vi "nominal_data_source.create.vi"(8 "error in":errorcluster, 9 "Description":string, 10 "Name":string, 11 "Nominal Client in":refnum<class "Nominal Client.lvclass">) -> (0 "error out":errorcluster, 1 "Created Data Source":T1, 2 "rid":string, 3 "Nominal Client out":refnum<class "Nominal Client.lvclass">)   [LabVIEW 2020, in "Nominal Client.lvclass"]
doc: "Creates a data source.\n\nid -> Required\nA human readable identifier. Must be unique within an organization. If the ID is not unique, a timestamp will be added to the ID.\n\ndescription -> Optional"
uses:
  Nominal Client.lvclass
  609118db-7d9c-428b-a577-7bf67d0e67c4.vi
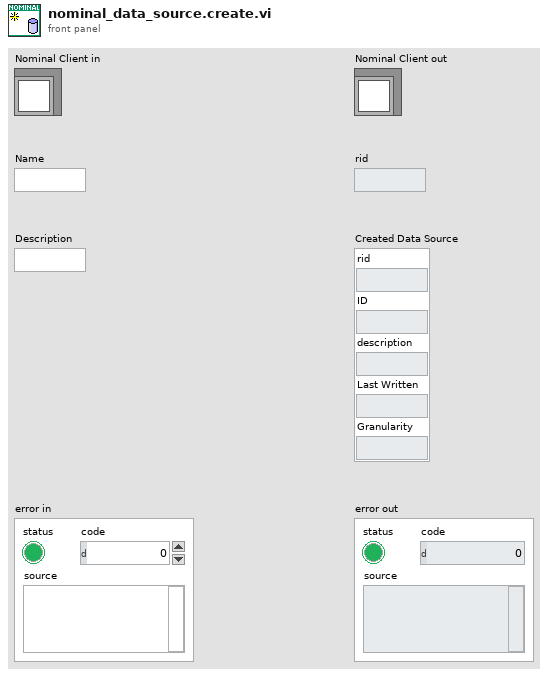
[diagram p1: front panel]
types:
  T1 = cluster{"rid":string, "ID":string, "description":string, "Last Written":string, "Granularity":string}
  T2 = cluster{"rid":string, "id":string, "description":string, "dataLastWrittenAt":string, "granularity":string}
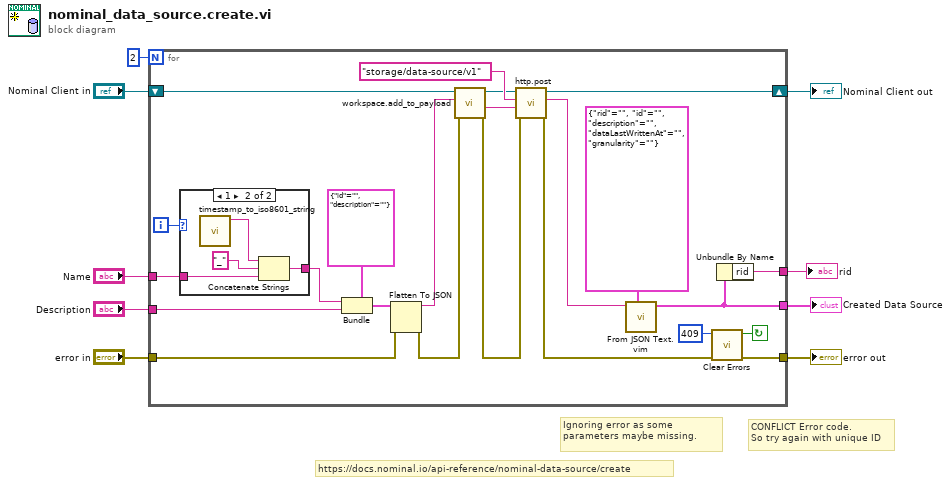
[diagram p0: block diagram]
diagram:
  # "CONFLICT Error code.\nSo try again with unique ID"
  # "Ignoring error as some parameters maybe missing."
  # "https://docs.nominal.io/api-reference/nominal-data-source/create"
  n1 = for {
    N: 2 -> [_]
    tunnel: "Name" -> [w21]
    tunnel: "Description" -> [w28]
    tunnel: [w24] -> w3
    tunnel: [w23] -> w2
    shift-right: [w32] -> w8
    shift-left: "Nominal Client in" -> [w15]
    tunnel: "error in" -> [w29]
    tunnel: [w17] -> w4
    i -> [w22]
    stop <- w16 continue-if-true
    n2 = case shown="1" w22 {
      tunnel: w21 -> [w33 w37]
      tunnel: [w33 w36] -> w20
      frame 0, Default {
      }
      frame 1 {
        n3 = call "timestamp_to_iso8601_string.vi"() -> ("ISO8601 UTC DateTime"=w34:string)  [unwired: 11 in]
        n4 = Concatenate Strings(w34, "_" ("string"), w37) -> (w36:string)
      }
    }
    n5 = Bundle(cluster=cluster{"id":string, "description":string} {"id"="", "description"=""}, "id"=w20, "description"=w28) -> (w30:cluster{"id":string, "description":string})
    n6 = Flatten To JSON(anything=w30, error in (no error)=w29) -> (JSON string=w14:string, 11:w11:errorcluster)  [unwired: 1 in]
    n7 = call "workspace.add_to_payload.vi"("error in"=w11, "JSON payload in"=w14, "Nominal Client in"=w15) -> ("error out"=w12:errorcluster, "JSON payload out"=w10:string, "Nominal Client out"=w13:refnum<class "Nominal Client.lvclass">)  [unwired: 6 in]
    n8 = call "http.post.vi"("error in"=w12, "Request body"=w10, "Path"="storage/data-source/v1", "Nominal Client in"=w13) -> ("error out"=w18:errorcluster, "Response"=w26:string, "Nominal Client out"=w32:refnum<class "Nominal Client.lvclass">)  [unwired: 4 in, 1 out]
    n9 = call "From JSON Text.vim"("Data Type and Default Value"=T2 {"rid"="", "id"="", "description"="", "dataLastWrittenAt"="", "granularity"=""}, "JSON"=w26) -> ("Data out"=w24:T2)  [unwired: 8 in, 1 out]
    n10 = call <vilib>:"Clear Errors.vi"("error in (no error)"=w18, "specific error code to clear (0: all)"=409) -> ("error out"=w17:errorcluster, "specific error cleared?"=w16:bool)  [unwired: 4 in]
    n11 = Unbundle By Name(w24) -> ("rid"=w23:string)
  }
  "Nominal Client out" <- w8
  "error out" <- w4
  "Created Data Source" <- w3
  "rid" <- w2
